vi "Run Server.vi"(8 "error in (no error)":errorcluster, 10 "NI GUID":string, 11 "Stop OOB Server UE":refnum<user-event>) -> (0 "error out":errorcluster)   [LabVIEW 2025, in "OOB gRPC Server.lvlib"]
uses:
  OOB gRPC Server.lvlib
  <vilib>/gRPC/LabVIEW gRPC Servicer/ServiceBase/ServiceBase.lvclass
  <vilib>/gRPC/LabVIEW gRPC Servicer/Servicer/Servicer.lvclass
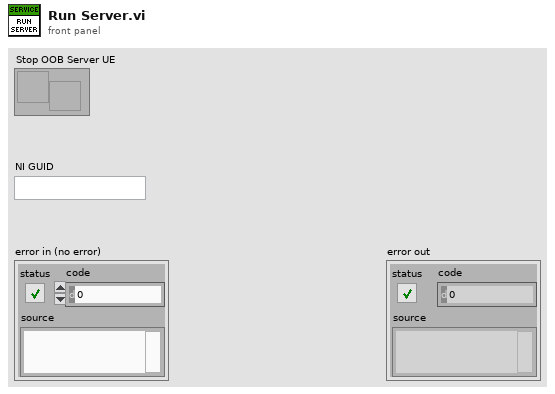
[diagram p1: front panel]
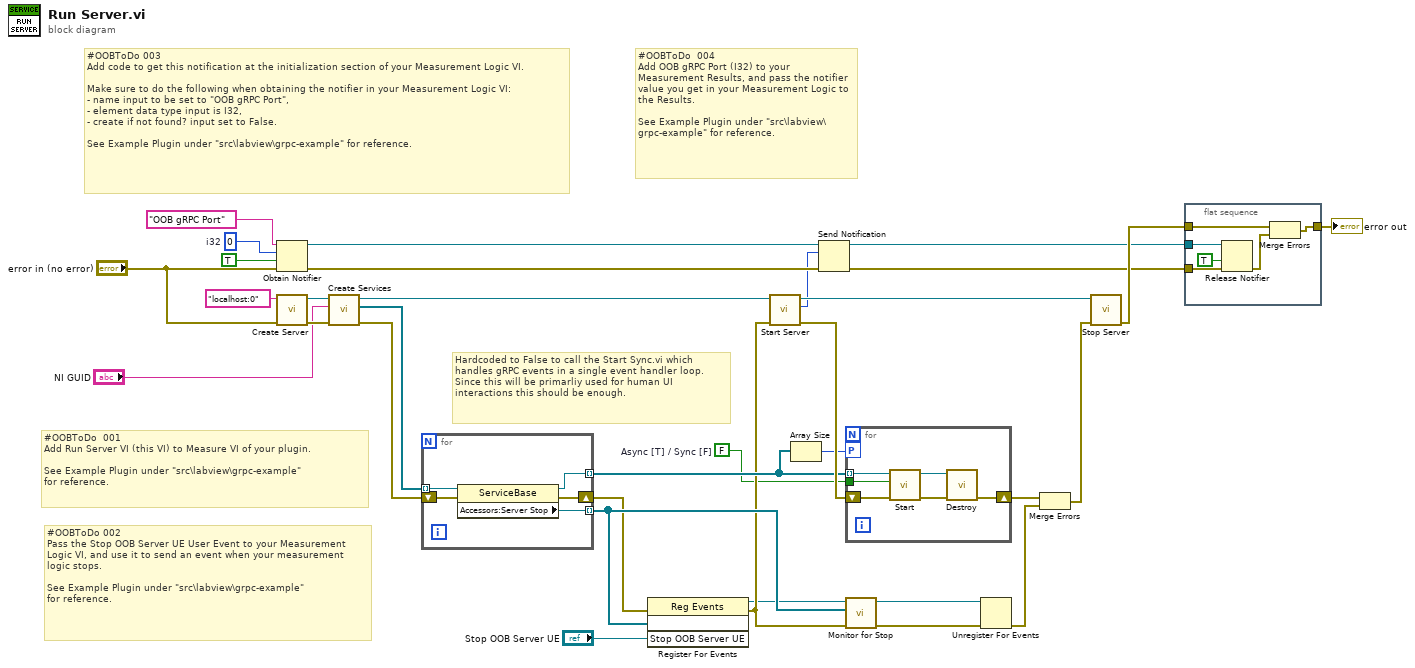
[diagram p0: block diagram]
diagram:
  w3 = FALSE  # Async [T] / Sync [F]
  w12 = 0  # i32
  # "#OOBToDo  004 \nAdd OOB gRPC Port (I32) to your Measurement Results, and pass the notifier value you get in your Measurement Logic to the Results.\n\nSee Example Plugin under \"src\\labview\\grpc-example\" for reference."
  # "#OOBToDo 002 \nPass the Stop OOB Server UE User Event to your Measurement Logic VI, and use it to send an event when your measurement logic stops.\n\nSee Example Plugin under \"src\\labview\\grpc-example\" for reference."
  # "#OOBToDo  001 \nAdd Run Server VI (this VI) to Measure VI of your plugin.\n\nSee Example Plugin under \"src\\labview\\grpc-example\" for reference."
  # "Hardcoded to False to call the Start Sync.vi which handles gRPC events in a single event handler loop.\nSince this will be primarliy used for human UI interactions this should be enough."
  # "#OOBToDo 003 \nAdd code to get this notification at the initialization section of your Measurement Logic VI. \n\nMake sure to do the following when obtaining the notifier in your Measurement Logic VI:\n- name input to be set to \"OOB gRPC Port\",\n- element data type input is I32,\n- create if not found? input set to False.\n\nSee Example Plugin under \"src\\labview\\grpc-example\" for reference."
  n1 = Obtain Notifier(name (unnamed)="OOB gRPC Port", notification data type=w12, create if not found? (T)=TRUE, error in (no error)="error in (no error)") -> (notifier out=w10:refnum<notifier>, error out=w9:errorcluster)  [unwired: 1 out]
  n2 = call <vilib>:"Create Server.vi"("error in"="error in (no error)", "Server Address"="localhost:0") -> ("error out"=w18:errorcluster, "gRPC server out"=w32:refnum<class "Servicer.lvclass">)  [unwired: 8 in]
  n3 = call "Create Services.vi"("error in (no error)"=w18, "NI GUID"="NI GUID", "gRPC server in"=w32) -> ("error out"=w17:errorcluster, "gRPC services out"=w16:refnum<class "ServiceBase.lvclass">[], "gRPC server out"=w31:refnum<class "Servicer.lvclass">)  [unwired: 6 in]
  n4 = for {
    tunnel: [w37] -> w27 mode=indexing
    shift-right: [w36] -> w26
    shift-left: w17 -> [w34]
    tunnel: [w38] -> w28 mode=indexing
    tunnel: w16 -> [w35] mode=indexing
    n5 = property class="ServiceBase"(reference=w35, error in=w34) -> (reference out=w38:refnum<class "ServiceBase.lvclass">, error out=w36:errorcluster, "Accessors:Server Stop"=w37:refnum<user-event>)
  }
  n6 = register-events(error in=w26, w27, "Stop OOB Server UE") -> (reference out=w2:refnum<event-registration>, error out=w25:errorcluster)  [unwired: 1 in]
  n7 = call <vilib>:"Start Server.vi"("error in"=w25, "gRPC server in"=w31) -> ("error out"=w30:errorcluster, "Listening Port"=w6:i32, "gRPC server out"=w33:refnum<class "Servicer.lvclass">)  [unwired: 7 in]
  n8 = Array Size(array=w28) -> (size(s)=w29:i32)
  n9 = Send Notification(notification=w6, notifier=w10, error in (no error)=w9) -> (notifier out=w5:refnum<notifier>, error out=w4:errorcluster)
  n10 = for {
    tunnel: w28 -> [w42] mode=indexing
    tunnel: w3 -> [w40]
    workers-P: w29 -> [_]
    shift-right: [w39] -> w24
    shift-left: w30 -> [w41]
    n11 = call-dynamic "Start.vi"("error in"=w41, "ASync [T]"=w40, "gRPC service in"=w42) -> ("error out"=w43:errorcluster, "gRPC service out"=w44:refnum<class "ServiceBase.lvclass">)  [unwired: 7 in]
    n12 = call-dynamic "Destroy.vi"("error in"=w43, "gRPC service in"=w44) -> ("error out"=w39:errorcluster)  [unwired: 8 in, 1 out]
  }
  n13 = call "Monitor for Stop.vi"("error in (no error)"=w25, "service stop events"=w27, "Event Registration Refnum in"=w2) -> ("error out"=w20:errorcluster, "Event Registration Refnum out"=w22:refnum<event-registration>)  [unwired: 7 in]
  n14 = Unregister For Events(event registration refnum=w22, error in=w20) -> (error out=w21:errorcluster)
  n15 = Merge Errors(w24, w21) -> (w23:errorcluster)
  n16 = call <vilib>:"Stop Server.vi"("error in"=w23, "gRPC server in"=w33) -> ("error out"=w19:errorcluster)  [unwired: 9 in]
  n17 = flat-sequence {
    tunnel: w5 -> [w50]
    tunnel: w19 -> [w48]
    tunnel: [w47] -> w14
    tunnel: w4 -> [w45]
    frame #0 {
      n18 = Release Notifier(notifier=w50, force destroy? (F)=TRUE, error in (no error)=w45) -> (error out=w46:errorcluster)  [unwired: 2 out]
      n19 = Merge Errors(w48, w46) -> (w47:errorcluster)
    }
  }
  "error out" <- w14
